vi "test_Add Custom Device.vi"(8 "error in (no error)":errorcluster, 11 "TestCase in":refnum<class "Scan Engine Scripting API Custom Device Unit Tests.lvclass">) -> (0 "error out":errorcluster, 3 "TestCase out":refnum<class "Scan Engine Scripting API Custom Device Unit Tests.lvclass">)   [LabVIEW 2027, in "Scan Engine Scripting API Custom Device Unit Tests.lvclass"]
uses:
  Scan Engine Scripting API Custom Device Unit Tests.lvclass
  Scan Engine Scripting API Custom Device Unit Tests.lvclass/Scan Engine Scripting API Custom Device Unit Tests.ctl
  <vilib>/addons/_JKI Toolkits/VI Tester/TestCase.llb/TestCase.lvclass
  Scripting/Scan Engine Scripting.lvlib
  Shared/Type Defs/Main Settings.ctl
  Shared/SEECD Shared.lvlib
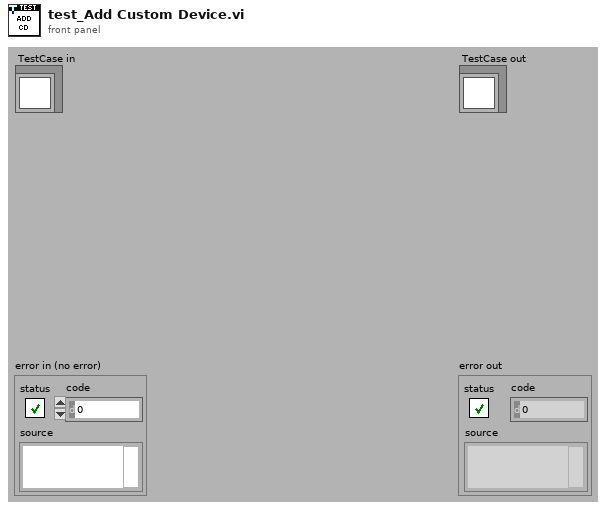
[diagram p1: front panel]
types:
  T1 = typedef "SEECD Shared.lvlib/Main Settings.ctl" = cluster{"sync to scan":bool, "scan engine decimation":u16, "delay after FPGA load (s)":u16}
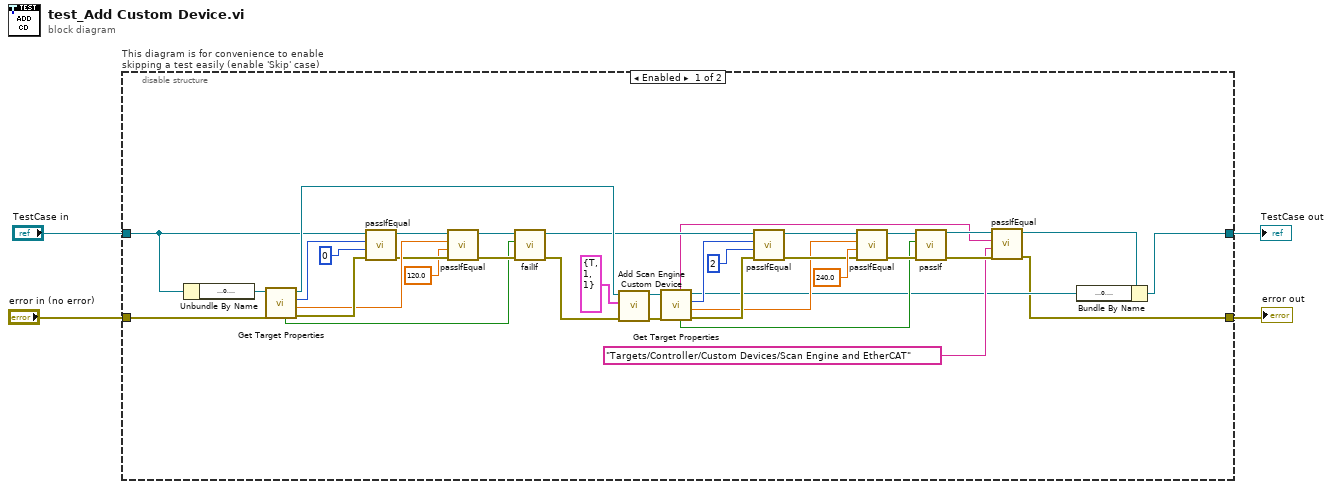
[diagram p0: block diagram]
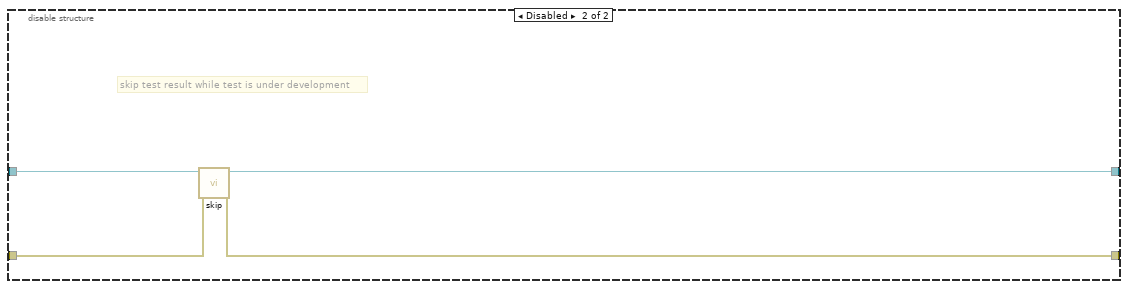
[diagram p2: hidden frame]
diagram:
  n1 = disable-structure "This diagram is for convenience to enable skipping a test easily (enable 'Skip' case)" shown="Enabled" {
    disable-tunnel: "TestCase in" -> [w11 w45]
    disable-tunnel: [w6 w43] -> w1
    disable-tunnel: [w5 w44] -> w3
    disable-tunnel: "error in (no error)" -> [w9 w42]
    frame Enabled {
      n2 = Unbundle By Name(w11) -> ("target ref"=w10:refnum<k24>)
      n3 = call "Get Target Properties.vi"("error in"=w9, "target ref in"=w10) -> ("error out"=w38:errorcluster, "TL timeout value"=w37:dbl, "ts value"=w40:u32, "target ref out"=w30:refnum<k24>, "dependent node found"=w12:bool)  [unwired: 4 in, 1 out]
      n4 = call-dynamic "passIfEqual.vi"("error in (no error)"=w38, "y"=u32 0 ("ts value"), "x"=w40, "TestCase in"=w11) -> ("error out"=w35:errorcluster, "TestCase out"=w36:refnum<class "Scan Engine Scripting API Custom Device Unit Tests.lvclass">)  [unwired: 6 in]
      n5 = call-dynamic "passIfEqual.vi"("error in (no error)"=w35, "y"=120.0 ("TL timeout value"), "x"=w37, "TestCase in"=w36) -> ("error out"=w33:errorcluster, "TestCase out"=w32:refnum<class "Scan Engine Scripting API Custom Device Unit Tests.lvclass">)  [unwired: 6 in]
      n6 = call-dynamic "failIf.vi"("error in (no error)"=w33, "fail"=w12, "TestCase in"=w32) -> ("error out"=w31:errorcluster, "TestCase out"=w19:refnum<class "Scan Engine Scripting API Custom Device Unit Tests.lvclass">)  [unwired: 7 in]
      n7 = call "Add Scan Engine Custom Device.vi"("error in"=w31, "settings"=T1 {"sync to scan"=TRUE, "scan engine decimation"=1, "delay after FPGA load (s)"=1}, "target in"=w30) -> ("error out"=w23:errorcluster, "target out"=w22:refnum<k24>)  [unwired: 6 in, 1 out]
      n8 = call "Get Target Properties.vi"("error in"=w23, "target ref in"=w22) -> ("error out"=w21:errorcluster, "TL timeout value"=w18:dbl, "ts value"=w20:u32, "target ref out"=w7:refnum<k24>, "dependent node found"=w17:bool, "dependent custom device node path"=w14:string)  [unwired: 4 in]
      n9 = call-dynamic "passIfEqual.vi"("error in (no error)"=w21, "y"=u32 2 ("ts value"), "x"=w20, "TestCase in"=w19) -> ("error out"=w26:errorcluster, "TestCase out"=w25:refnum<class "Scan Engine Scripting API Custom Device Unit Tests.lvclass">)  [unwired: 6 in]
      n10 = call-dynamic "passIfEqual.vi"("error in (no error)"=w26, "y"=240.0 ("TL timeout value"), "x"=w18, "TestCase in"=w25) -> ("error out"=w28:errorcluster, "TestCase out"=w29:refnum<class "Scan Engine Scripting API Custom Device Unit Tests.lvclass">)  [unwired: 6 in]
      n11 = call-dynamic "passIf.vi"("error in (no error)"=w28, "pass"=w17, "TestCase in"=w29) -> ("error out"=w16:errorcluster, "TestCase out"=w15:refnum<class "Scan Engine Scripting API Custom Device Unit Tests.lvclass">)  [unwired: 7 in]
      n12 = call-dynamic "passIfEqual.vi"("error in (no error)"=w16, "y"="Targets/Controller/Custom Devices/Scan Engine and EtherCAT", "x"=w14, "TestCase in"=w15) -> ("error out"=w5:errorcluster, "TestCase out"=w8:refnum<class "Scan Engine Scripting API Custom Device Unit Tests.lvclass">)  [unwired: 6 in]
      n13 = Bundle By Name(cluster=w8, "target ref"=w7) -> (w6:refnum<class "Scan Engine Scripting API Custom Device Unit Tests.lvclass">)
    }
    frame Disabled {
      # "skip test result while test is under development"
      n14 = call <vilib>:"skip.vi"("error in (no error)"=w42, "TestCase in"=w45) -> ("error out"=w44:errorcluster, "TestCase out"=w43:refnum<class "Scan Engine Scripting API Custom Device Unit Tests.lvclass">)  [unwired: 8 in]
    }
  }
  "error out" <- w3
  "TestCase out" <- w1
